vi "POST HTTP Literal.vi"(11 "error in":errorcluster) -> (15 "error out":errorcluster)   [LabVIEW 2024]
doc: "Static analysis fixture for a POSTBuffer call with an HTTP literal. A constant-false selector disables the call."
uses:
  <vilib>/httpClient/LabVIEWHTTPClient.lvlib
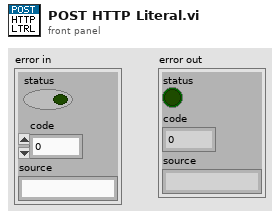
[diagram p1: front panel]
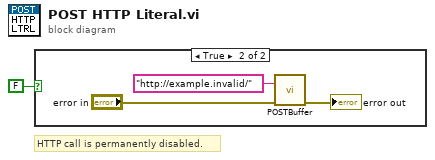
[diagram p0: block diagram]
diagram:
  # "HTTP call is permanently disabled."
  n1 = case shown="True" FALSE ("guard") {
    frame False {
    }
    frame True {
      n2 = call <vilib>:"POSTBuffer.vi"("url"="http://example.invalid/", "error in (no error)"="error in") -> ("error out"=→"error out":errorcluster)  [unwired: 10 in, 3 out]
    }
  }
